vi "F3_Append_Line.vi"(10 "Value":dbl, 11 "File Path":path) -> (2 "error out":errorcluster, 3 "Line":string)   [LabVIEW 2026]
doc: "Use this template to build a VI to use as a subVI."
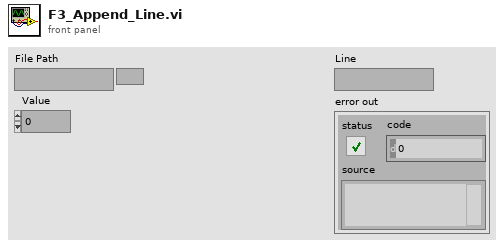
[diagram p1: front panel]
types:
  T1 = enum16{"open", "replace", "create", "open or create", "replace or create", "replace or create with confirmation"}
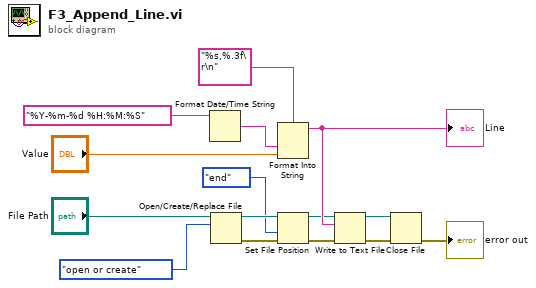
[diagram p0: block diagram]
diagram:
  n1 = Format Date/Time String(time format string (%c)="%Y-%m-%d %H:%M:%S") -> (date/time string=w8:string)  [unwired: 2 in]
  n2 = Open/Create/Replace File(file path (use dialog)="File Path", operation (0:open)=T1."open or create") -> (refnum out=w13:refnum<file>, error out=w12:errorcluster)  [unwired: 4 in, 1 out]
  n3 = Format Into String(format string="%s,%.3f\r\n", w8, "Value") -> (resulting string=w6:string)  [unwired: 2 in, 1 out]
  "Line" <- w6
  n4 = Set File Position(refnum=w13, from (0:start)=enum16{"start", "end", "current"}."end", error in=w12) -> (refnum out=w5:refnum<file>, error out=w4:errorcluster)  [unwired: 1 in]
  n5 = Write to Text File(file (use dialog)=w5, text=w6, error in=w4) -> (refnum out=w3:refnum<file>, error out=w2:errorcluster)  [unwired: 1 in, 1 out]
  n6 = Close File(refnum=w3, error in=w2) -> (error out=→"error out":errorcluster)  [unwired: 1 out]
